vi "RemoteVI Post Input.vi"(0 "hWnd":u64, 1 "popup since":u32, 5 "posts":cluster{"msg":u32, "wParam":u64, "lParam":i64}[](array[cluster]), 7 "cursor":cluster{"move?":bool, "x":i32, "y":i32}, 9 "popups":T1, 11 "error in":errorcluster) -> (4 "popups out":T1, 15 "error out":errorcluster)   [LabVIEW 2020, in "RemoteVI.lvlib"]
doc: "Posts the Win32 messages from RemoteVI Translate Input.vi to the window hWnd (the served front panel), in order, with user32 PostMessageW. First RemoteVI Swallow Button Up.vi drops the button-up of a click that was turned into menu keys. Without a popup (cursor.move? FALSE) each message is posted only after LabVIEW has handled the one before - except after a hover move (WM_MOUSEMOVE with no button held), which nothing waits on; at up to 60 moves per second the round trips kept the server loop waiting for LabVIEW's busy UI thread (measured on the demo) - : after every other PostMessageW the VI waits with RemoteVI Wait Input Handled.vi (two WM_NULL sent to hWnd, at most 500 ms each) - LabVIEW drops and reorders key messages that arrive in a burst (measured: twelve posted Backspace key-downs became one), and the server decides how to post a button-up from the mouse capture the button-down set up. With a popup open (cursor.move? TRUE, a button message at the LOGICAL screen point cursor.x, cursor.y) the message goes to RemoteVI Popup Click.vi (docs\\architecture.md, Popups): on a LabVIEW menu it is done with keys (VK_LEFT, VK_DOWN / VK_UP, VK_RETURN) - no menu and no cursor moves, so every submenu opens where LabVIEW opens it locally; on a popup that takes no keys (colour picker, line width popup, graph palette popups) only that window is moved under the host cursor for the message and moved back; outside every popup a button-down closes them all (WM_CANCELMODE). The host cursor never moves. popups passes through to popups out unchanged (the displacement d stays 0: popups are no longer left displaced). No VI Server call, so it works while an open popup blocks LabVIEW's UI thread. An incoming error posts nothing."
uses:
  RemoteVI.lvlib
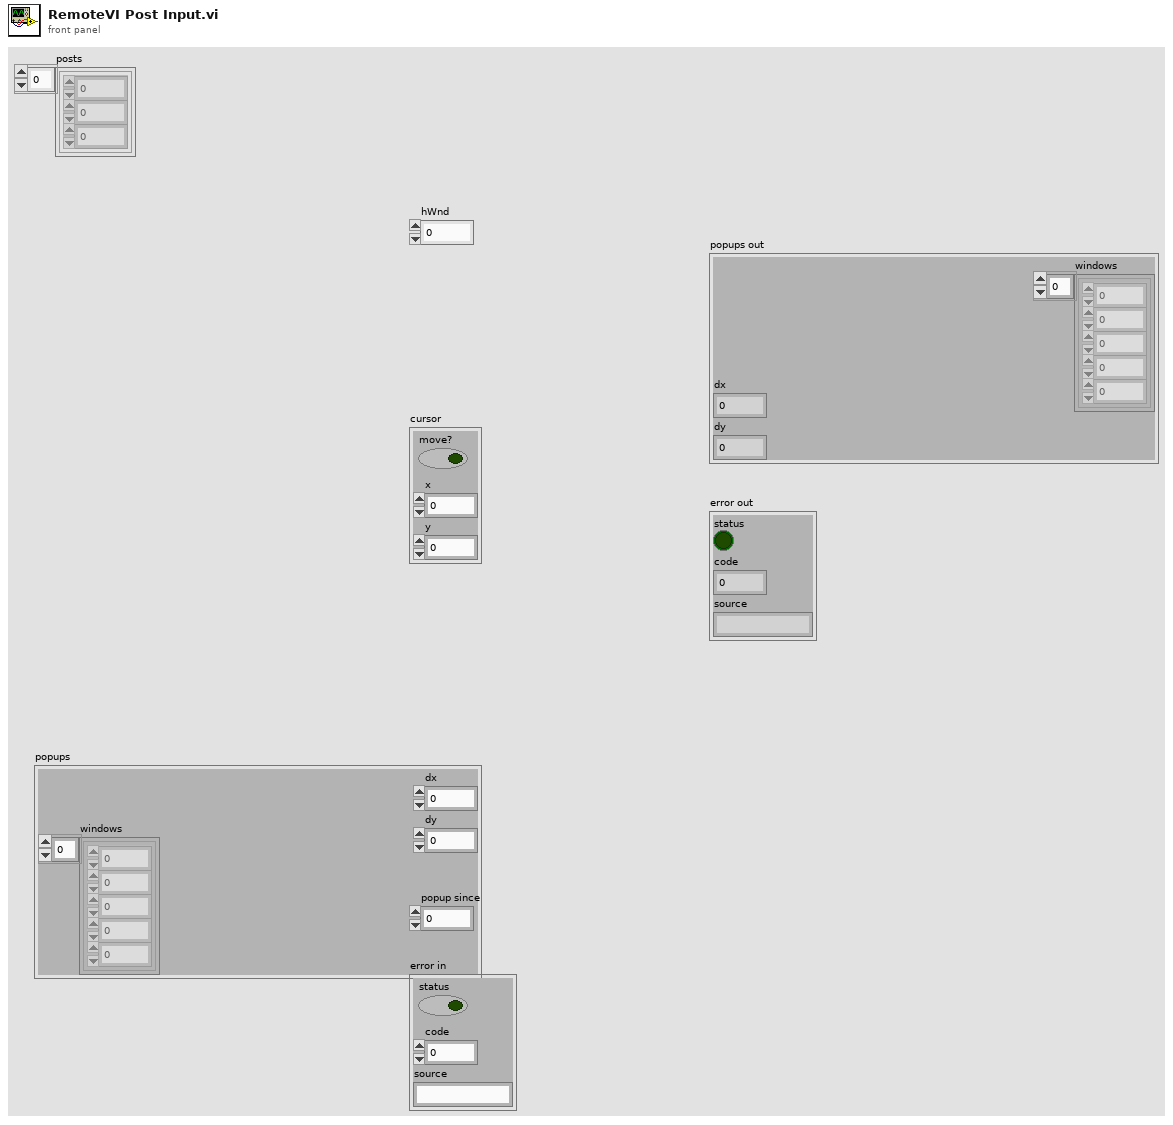
[diagram p1: front panel]
types:
  T1 = cluster{"windows":cluster{"hwnd":u64, "x":i32, "y":i32, "w":i32, "h":i32}[], "dx":i32, "dy":i32}
  T2 = cluster{"hwnd":u64, "x":i32, "y":i32, "w":i32, "h":i32}[]
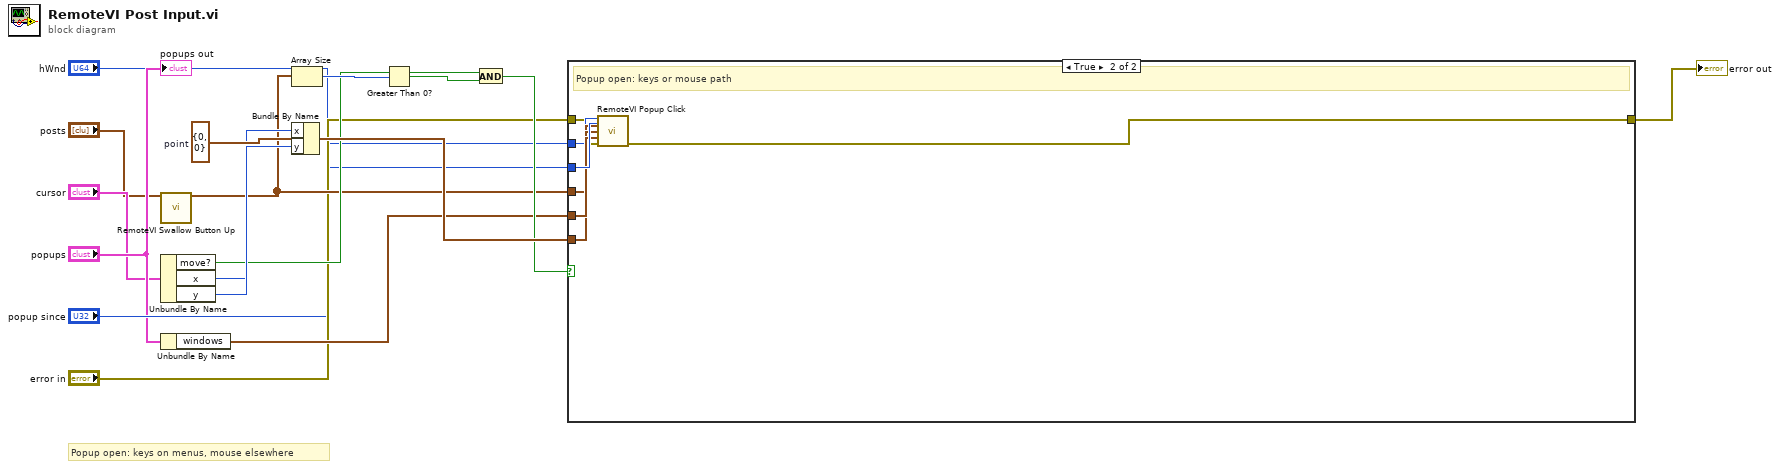
[diagram p0: block diagram]
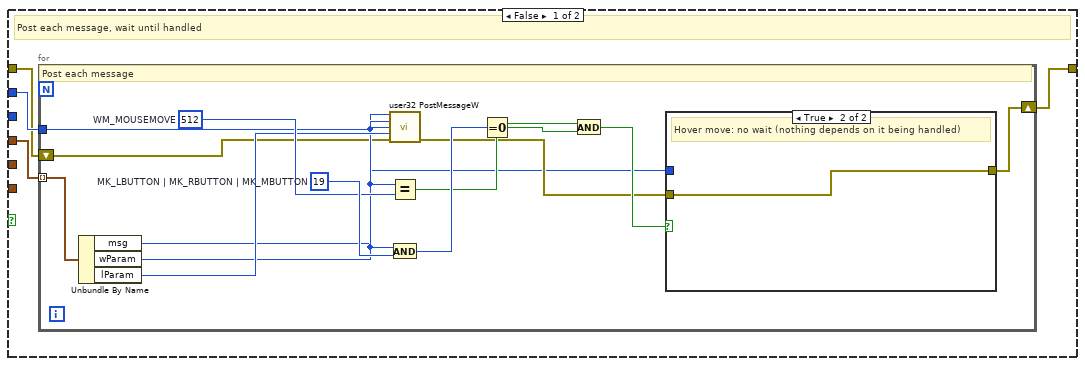
[diagram p2: hidden frame]
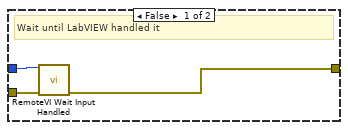
[diagram p3: hidden frame]
diagram:
  w15 = cluster{"x":i32, "y":i32} {"x"=0, "y"=0}  # point
  # "Popup open: keys on menus, mouse elsewhere"
  n1 = call "RemoteVI Swallow Button Up.vi"("posts"="posts") -> ("posts out"=w7:cluster{"msg":u32, "wParam":u64, "lParam":i64}[])  [unwired: 14 in]
  n2 = Unbundle By Name("cursor") -> ("move?"=w8:bool, "x"=w9:i32, "y"=w10:i32)
  n3 = Unbundle By Name("popups") -> ("windows"=w11:T2)
  n4 = Array Size(array=w7) -> (size(s)=w12:i32)
  n5 = Bundle By Name(cluster=w15, "x"=w9, "y"=w10) -> (w16:cluster{"x":i32, "y":i32})
  n6 = Greater Than 0?(x=w12) -> (x > 0?=w13:bool)
  n7 = And(x=w8, y=w13) -> (x .and. y?=w14:bool)
  n8 = case shown="True" w14 {
    tunnel: "error in" -> [w18 w40]
    tunnel: "hWnd" -> [w19 w41]
    tunnel: "popup since" -> [_ w45]
    tunnel: w7 -> [w20 w42]
    tunnel: w11 -> [_ w44]
    tunnel: w16 -> [_ w43]
    tunnel: [w21 w46] -> w17
    frame False {
      # "Post each message, wait until handled"
      n9 = for {
        tunnel: w19 -> [w23]
        shift-right: [w25] -> w21
        shift-left: w18 -> [w24]
        tunnel: w20 -> [w22] mode=indexing
        w31 = u64 19  # MK_LBUTTON | MK_RBUTTON | MK_MBUTTON
        w30 = u32 512  # WM_MOUSEMOVE
        # "Post each message"
        n10 = Unbundle By Name(w22) -> ("msg"=w26:u32, "wParam"=w27:u64, "lParam"=w28:i64)
        n11 = call "user32 PostMessageW.vi"("hWnd"=w23, "Msg"=w26, "wParam"=w27, "lParam"=w28, "error in (no error)"=w24) -> ("error out"=w29:errorcluster)  [unwired: 9 in, 1 out]
        n12 = Equal?(x=w26, y=w30) -> (x = y?=w32:bool)
        n13 = And(x=w27, y=w31) -> (x .and. y?=w33:u64)
        n14 = Equal To 0?(x=w33) -> (x = 0?=w34:bool)
        n15 = And(x=w32, y=w34) -> (x .and. y?=w35:bool)
        n16 = case shown="True" w35 {
          tunnel: w23 -> [w36 _]
          tunnel: w29 -> [w37 w39]
          tunnel: [w38 w39] -> w25
          frame False {
            # "Wait until LabVIEW handled it"
            n17 = call "RemoteVI Wait Input Handled.vi"("hWnd"=w36, "error in"=w37) -> ("error out"=w38:errorcluster)  [unwired: 13 in]
          }
          frame True {
            # "Hover move: no wait (nothing depends on it being handled)"
          }
        }
      }
    }
    frame True {
      # "Popup open: keys or mouse path"
      n18 = call "RemoteVI Popup Click.vi"("hWnd"=w41, "popup since"=w45, "posts"=w42, "point"=w43, "windows"=w44, "error in"=w40) -> ("error out"=w46:errorcluster)  [unwired: 9 in]
    }
  }
  "error out" <- w17
  "popups out" <- "popups"
